vi "Add Conformance Fixtures.vi"(8 "error in":errorcluster, 11 "server id":i32) -> (0 "error out":errorcluster, 3 "server id out":i32)   [LabVIEW 2020, in "Conformance MCP Server.lvlib"]
doc: "Registers everything the official MCP conformance suite calls by a fixed name on an MCP server: the tool VIs in the folder tools and the prompt VIs in the folder prompts beside this VI (the VI file name is the tool or prompt name), and the files static-text.txt and static-binary.png beside this VI as the resources test://static-text and test://static-binary. With an error coming in nothing is registered."
uses:
  Conformance MCP Server.lvlib
  src/MCP Server/MCP Server.lvlib
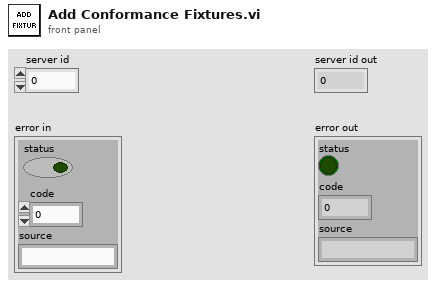
[diagram p1: front panel]
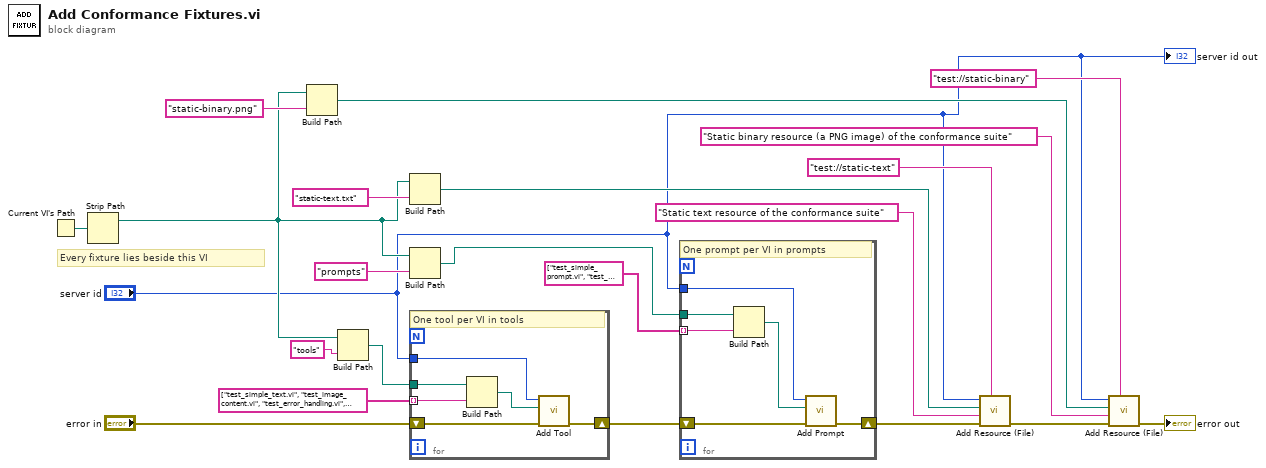
[diagram p0: block diagram]
diagram:
  # "Every fixture lies beside this VI"
  n1 = Current VI's Path() -> (path=w3:path)
  n2 = Strip Path(path=w3) -> (stripped path=w4:path)  [unwired: 1 out]
  n3 = Build Path(base path=w4, name or relative path="static-binary.png" ("file")) -> (appended path=w21:path)
  n4 = Build Path(base path=w4, name or relative path="tools" ("tools folder")) -> (appended path=w6:path)
  n5 = Build Path(base path=w4, name or relative path="static-text.txt" ("file")) -> (appended path=w16:path)
  n6 = Build Path(base path=w4, name or relative path="prompts" ("prompts folder")) -> (appended path=w10:path)
  n7 = for {
    tunnel: string[] ["test_simple_text.vi", "test_image_content.vi", "test_error_handling.vi", "test_tool_with_progress.vi", "test_input_required_result_elicitation.vi", "test_input_required_result_request_state.vi", "test_input_required_result_multi_round.vi", "test_input_required_result_tampered_state.vi"] ("tools VIs") -> [w23] mode=indexing
    tunnel: "server id" -> [w25]
    shift-right: [w27] -> w8
    shift-left: "error in" -> [w28]
    tunnel: w6 -> [w24]
    # "One tool per VI in tools"
    n8 = Build Path(base path=w24, name or relative path=w23) -> (appended path=w26:path)
    n9 = call "Add Tool.vi"("error in (no error)"=w28, "vi path"=w26, "server id"=w25) -> ("error out"=w27:errorcluster)  [unwired: 7 in, 1 out]
  }
  n10 = for {
    tunnel: string[] ["test_simple_prompt.vi", "test_prompt_with_arguments.vi", "test_input_required_result_prompt.vi"] ("prompts VIs") -> [w29] mode=indexing
    tunnel: "server id" -> [w31]
    shift-right: [w33] -> w12
    shift-left: w8 -> [w34]
    tunnel: w10 -> [w30]
    # "One prompt per VI in prompts"
    n11 = Build Path(base path=w30, name or relative path=w29) -> (appended path=w32:path)
    n12 = call "Add Prompt.vi"("error in (no error)"=w34, "vi path"=w32, "server id"=w31) -> ("error out"=w33:errorcluster)  [unwired: 7 in, 1 out]
  }
  n13 = call "Add Resource (File).vi"("uri"="test://static-text", "error in (no error)"=w12, "description"="Static text resource of the conformance suite", "file path"=w16, "server id"="server id") -> ("error out"=w17:errorcluster)  [unwired: 5 in, 1 out]
  n14 = call "Add Resource (File).vi"("uri"="test://static-binary", "error in (no error)"=w17, "description"="Static binary resource (a PNG image) of the conformance suite", "file path"=w21, "server id"="server id") -> ("error out"=→"error out":errorcluster)  [unwired: 5 in, 1 out]
  "server id out" <- "server id"
